vi "Generate Trace for Connected Network Endpoint.vi"(8 "error in":errorcluster, 9 "Port":string, 10 "IP or Stream Name":string) -> ()   [LabVIEW 2020]
doc: "Generates a DETT User Generated Trace for a network endpoint being connected to other one."
uses:
  <resource>/AFDebug/AF Debug.lvlib
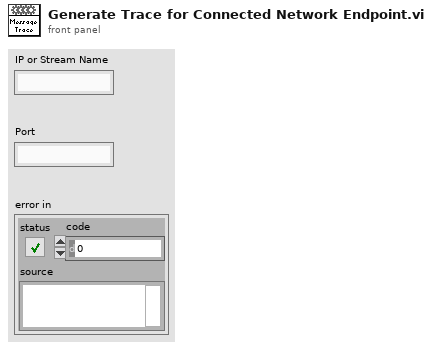
[diagram p1: front panel]
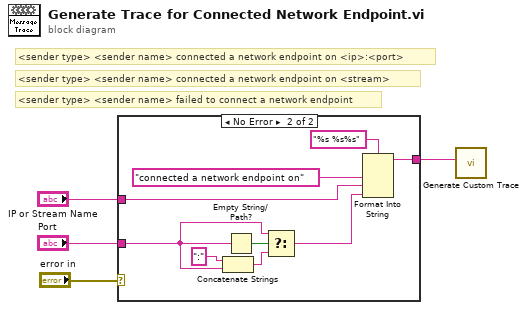
[diagram p0: block diagram]
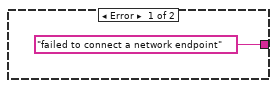
[diagram p2: hidden frame]
diagram:
  # "<sender type> <sender name> connected a network endpoint on <stream>"
  # "<sender type> <sender name> failed to connect a network endpoint"
  # "<sender type> <sender name> connected a network endpoint on <ip>:<port>"
  n1 = case shown="No Error" "error in" {
    tunnel: "Port" -> [_ w7]
    tunnel: ["failed to connect a network endpoint" ("input 3") w11] -> w2
    tunnel: "IP or Stream Name" -> [_ w14]
    frame Error {
    }
    frame No Error {
      n2 = Concatenate Strings(":" ("string"), w7) -> (w8:string)
      n3 = Empty String/Path?(string/path=w7) -> (empty?=w9:bool)
      n4 = Select(t=w7, s=w9, f=w8) -> (s? t:f=w6:string)
      n5 = Format Into String(format string="%s %s%s", "connected a network endpoint on" ("input 3"), w14, w6) -> (resulting string=w11:string)  [unwired: 2 in, 1 out]
    }
  }
  n6 = call <resource>:"Generate Custom Trace.vi"("Custom Action"=w2) -> ()  [unwired: 11 in]
